vi "Initialize From Config.vi"(8 "error in":errorcluster, 9 "Module Configurations":refnum<class "TBM module configuration.lvclass">[](array[class]), 10 "Modules":refnum<class "TBM module execution interface.lvclass">[](array[class]), 11 "Engine Configuration":refnum<class "synchronous engine configuration.lvclass">) -> (0 "error out":errorcluster, 3 "Engine Data Out":T1={"Main Tag Data"={"Double"=[], "Single"=[], "I64"=[], "I32"=[], "I16"=[], "I8"=[], "U64"=[], "U32"=[], "U16"=[], "U8"=[], "Boolean"=[], "String"=[], "Array of Double"=[], "Array of Single"=[], "Array of I64"=[], "Array of I32"=[], "Array of I16"=[], "Array of I8"=[], "Array of U64"=[], "Array of U32"=[], "Array of U16"=[], "Array of U8"=[], "Array of Boolean"=[], "Array of String"=[]}, "Module Info"={"Tag Bus Modules"=[], "Input Method Indices"=[], "Process Method Indices"=[], "Output Method Indices"=[], "Input Transfer Specifications"=[], "Parameter Transfer Specifications"=[], "Result Transfer Specifications"=[], "Output Transfer Specifications"=[], "Module Errors"=[], "UID"=""}, "Safe State?"=FALSE, "engine timing source"=refnum, "Processor"=5000, "Priority"=-2, "dT"=0})   [LabVIEW 2014, in "synchronous engine runtime.lvclass"]
uses:
  synchronous engine runtime.lvclass
  Engine Data.ctl
  <vilib>/NI/Module Timing Source/timing source/TBM timing source.lvclass
  <vilib>/NI/Tag Bus/table/data table.ctl
  Module Execution Info.ctl
  <vilib>/NI/Tag Bus Module Framework/runtime/TBM module execution interface.lvclass
  Data Table with Transfer Spec.ctl
  <vilib>/NI/Tag Bus/table/transfer specification.ctl
  <vilib>/NI/Tag Bus/tag/Data Type.ctl
  Configuration/synchronous engine configuration.lvclass
  <vilib>/NI/Tag Bus Module Framework/module configuration/TBM module configuration.lvclass
  <vilib>/NI/Module Timing Source/usec timing source/usec timing source.lvclass
  Configuration/synchronous engine configuration.lvclass/synchronous engine configuration.ctl
  Engine Configuration/engine configuration.lvclass/engine configuration.ctl
  <vilib>/NI/Tag Bus/dictionary/data dictionary.lvclass/data dictionary.ctl
  <vilib>/NI/Configuration Framework/serializable configuration/NISE_CEF_serializable configuration.lvclass/NISE_CEF_serializable configuration.ctl
  <vilib>/NI/Configuration Framework/serializable configuration/Read UID.vi
  Configuration/Read Processor.vi
  Configuration/Read Priority.vi
  Configuration/Read Timing Source dt.vi
  <vilib>/Utility/LVClass/Get LV Class Name.vi
  <vilib>/NI/Configuration Framework/error generator/NISE_error generator.vi
  <vilib>/NI/Tag Bus/dictionary/data dictionary.lvclass
  Engine Configuration/engine configuration.lvclass
  <vilib>/NI/Tag Bus/table/data table.lvlib
  <vilib>/NI/Tag Bus/tag/tag descriptor.lvclass
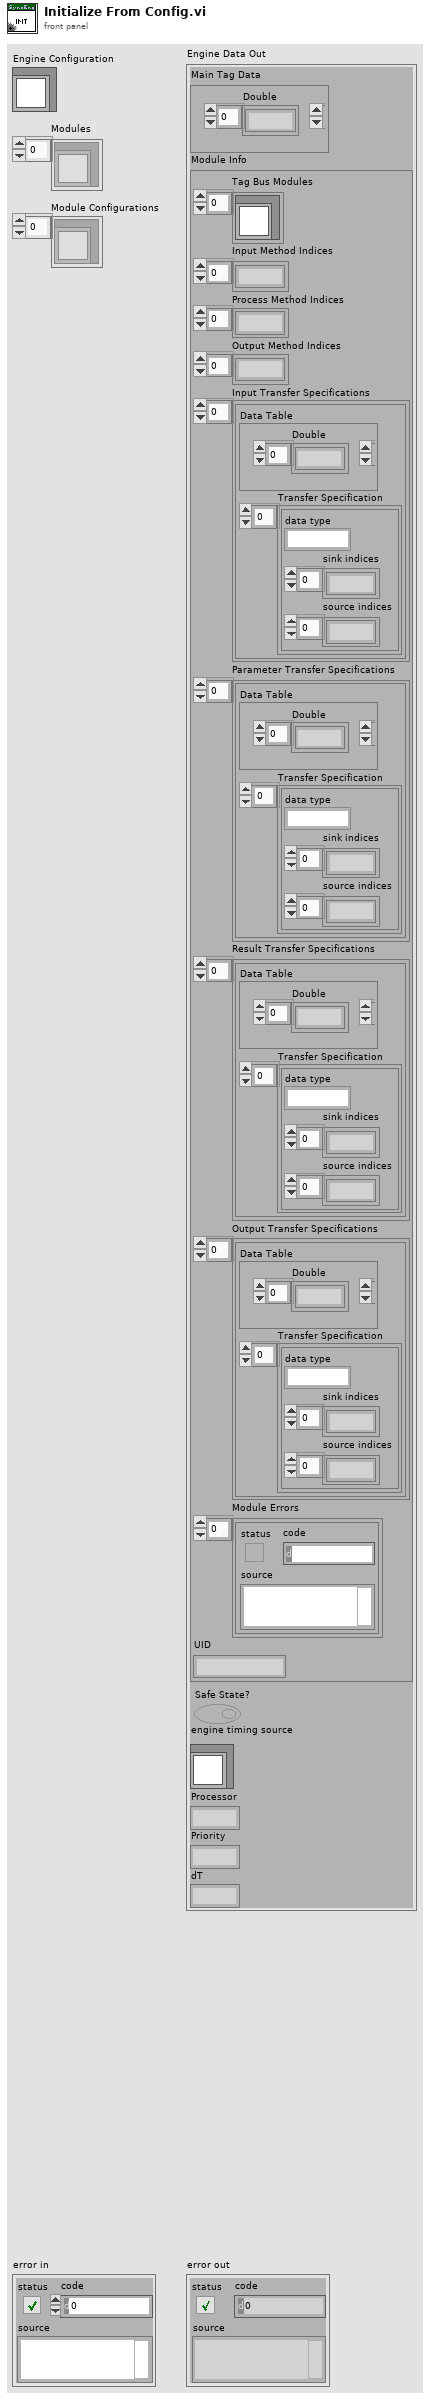
[diagram p1: front panel]
types:
  T1 = typedef "synchronous engine runtime.lvclass/Engine Data.ctl" = cluster{"Main Tag Data":T2, "Module Info":T3, "Safe State?":bool, "engine timing source":refnum<class "TBM timing source.lvclass">, "Processor":i32, "Priority":i32, "dT":u32}
  T2 = typedef "tag bus.lvlib/data table.lvlib/data table.ctl" = cluster{"Double":dbl[], "Single":sgl[], "I64":i64[], "I32":i32[], "I16":i16[], "I8":i8[], "U64":u64[], "U32":u32[], "U16":u16[], "U8":u8[], "Boolean":bool[], "String":string[], "Array of Double":cluster{"DBL Array":dbl[]}[], "Array of Single":cluster{"SGL Array":sgl[]}[], "Array of I64":cluster{"I64 Array":i64[]}[], "Array of I32":cluster{"I32 Array":i32[]}[], "Array of I16":cluster{"I16 Array":i16[]}[], "Array of I8":cluster{"I8 Array":i8[]}[], "Array of U64":cluster{"U64 Array":u64[]}[], "Array of U32":cluster{"U32 Array":u32[]}[], "Array of U16":cluster{"U16 Array":u16[]}[], "Array of U8":cluster{"U8 Array":u8[]}[], "Array of Boolean":cluster{"Boolean Array":bool[]}[], "Array of String":cluster{"String Array":string[]}[]}
  T3 = typedef "synchronous engine runtime.lvclass/Module Execution Info.ctl" = cluster{"Tag Bus Modules":refnum<class "TBM module execution interface.lvclass">[], "Input Method Indices":i32[], "Process Method Indices":i32[], "Output Method Indices":i32[], "Input Transfer Specifications":T4[], "Parameter Transfer Specifications":T4[], "Result Transfer Specifications":T4[], "Output Transfer Specifications":T4[], "Module Errors":errorcluster[], "UID":string}
  T4 = typedef "synchronous engine runtime.lvclass/Data Table with Transfer Spec.ctl" = cluster{"Data Table":T2, "Transfer Specification":T5[]}
  T5 = typedef "tag bus.lvlib/data table.lvlib/transfer specification.ctl" = cluster{"data type":T6, "sink indices":i32[], "source indices":i32[]}
  T6 = typedef "tag bus.lvlib/tag descriptor.lvclass/Data Type.ctl" = enum16{"Double", "Single", "I64", "I32", "I16", "I8", "U64", "U32", "U16", "U8", "Boolean", "String", "Array of Double", "Array of Single", "Array of I64", "Array of I32", "Array of I16", "Array of I8", "Array of U64", "Array of U32", "Array of U16", "Array of U8", "Array of Boolean", "Array of String"}
  T7 = typedef "TBM channel.lvclass/data tables.ctl" = cluster{"input data":T8, "processing parameter":T8, "processing result":T8, "output data":T8}
  T8 = typedef "tag bus.lvlib/dictionary table pair.ctl" = cluster{"data dictionary":refnum<class "data dictionary.lvclass">, "data table":T2}
  T9 = typedef "TBM module execution interface.lvclass/execution settings.ctl" = cluster{"reads inputs":bool, "processes data":bool, "writes outputs":bool}
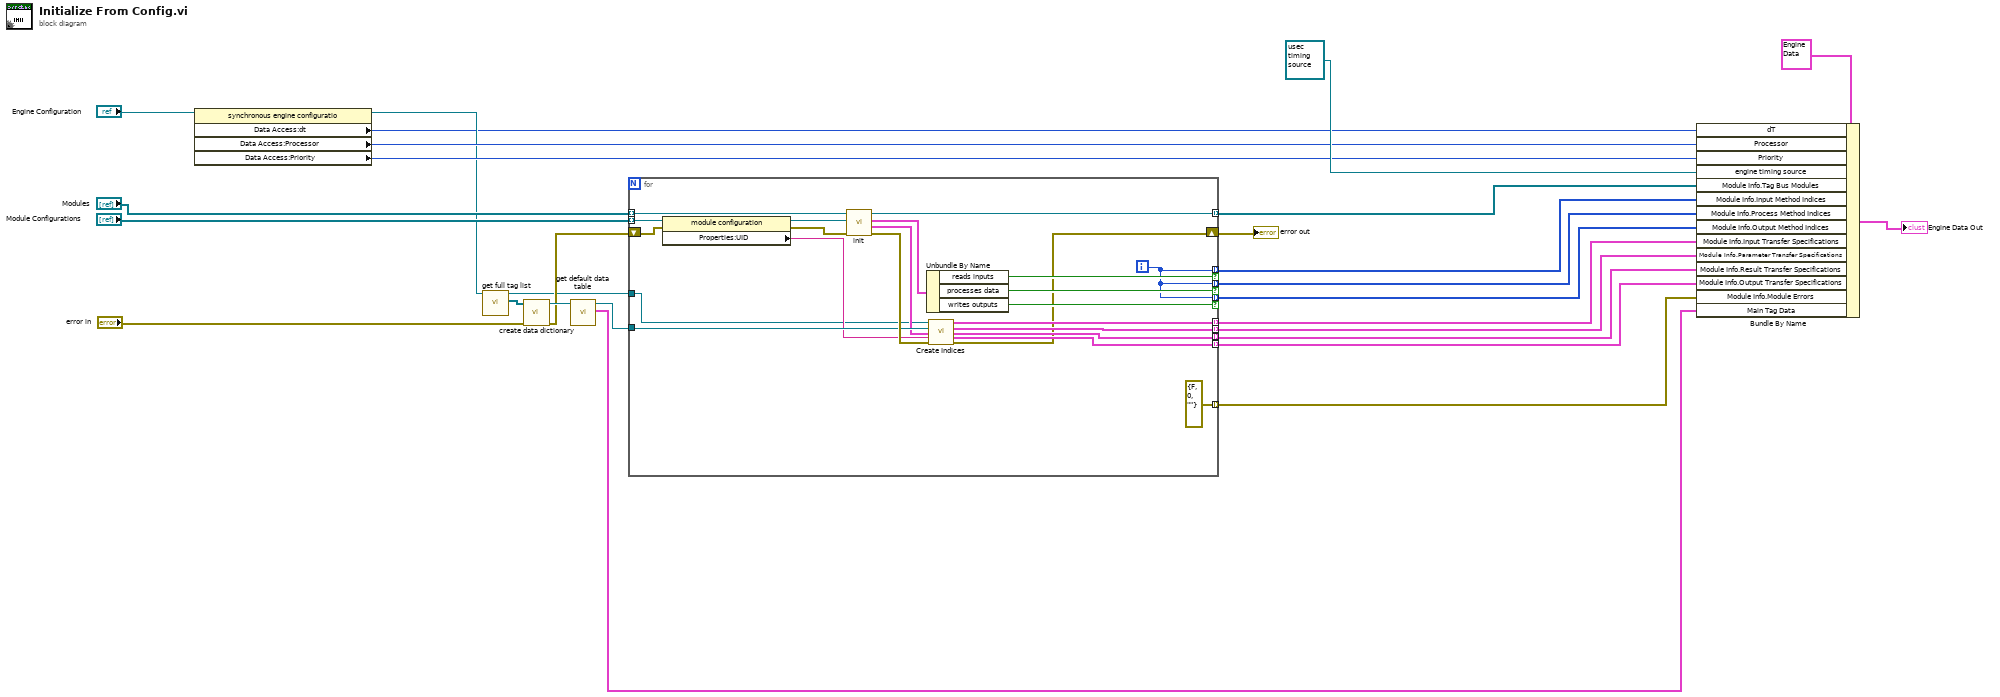
[diagram p0: block diagram]
diagram:
  n1 = property class="synchronous engine configuratio"(reference="Engine Configuration") -> (reference out=w2:refnum<class "synchronous engine configuration.lvclass">, "Data Access:dt"=w1:u32, "Data Access:Processor"=w4:i32, "Data Access:Priority"=w3:i32)  [unwired: 1 in, 1 out]
  n2 = call "get full tag list.vi"("engine configuration in"=w2) -> ("tag list"=w10:refnum<class "tag descriptor.lvclass">[], "engine configuration out"=w7:refnum<class "synchronous engine configuration.lvclass">)  [unwired: 9 in]
  n3 = call <vilib>:"create data dictionary.vi"("error in"="error in", "system tags"=w10) -> ("error out"=w8:errorcluster, "data dictionary"=w9:refnum<class "data dictionary.lvclass">)  [unwired: 8 in]
  n4 = call <vilib>:"get default data table.vi"("data dictionary in"=w9) -> ("default data table"=w16:T2, "data dictionary out"=w15:refnum<class "data dictionary.lvclass">)  [unwired: 9 in]
  n5 = for {
    tunnel: "Module Configurations" -> [w35] mode=indexing
    shift-right: [w30] -> w18
    shift-left: w8 -> [w32]
    tunnel: "Modules" -> [w49] mode=indexing
    tunnel: [w31] -> w27 mode=indexing
    tunnel: [w40] -> w25 mode=indexing if=w48
    tunnel: [w40] -> w24 mode=indexing if=w47
    tunnel: [w40] -> w23 mode=indexing if=w46
    tunnel: [w45] -> w22 mode=indexing
    tunnel: [w44] -> w21 mode=indexing
    tunnel: [w43] -> w20 mode=indexing
    tunnel: [w42] -> w19 mode=indexing
    tunnel: [errorcluster {"status"=FALSE, "code"=0, "source"=""} ("error constant")] -> w17 mode=indexing
    tunnel: w15 -> [w38]
    tunnel: w7 -> [w28]
    i -> [w40]
    n6 = property class="module configuration"(reference=w35, error in=w32) -> (reference out=w34:refnum<class "TBM module configuration.lvclass">, error out=w33:errorcluster, "Properties:UID"=w29:string)
    n7 = call-dynamic "init.vi"("error in"=w33, "module configuration"=w34, "module in"=w49) -> ("error out"=w41:errorcluster, "data allocations"=w36:T7, "execution settings"=w37:T9, "module out"=w31:refnum<class "TBM module execution interface.lvclass">)  [unwired: 5 in]
    n8 = Unbundle By Name(w37) -> ("reads inputs"=w48:bool, "processes data"=w47:bool, "writes outputs"=w46:bool)
    n9 = call "Create Indices.vi"("synchronous engine configuration"=w28, "main data dictionary"=w38, "data description"=w36, "Module ID"=w29, "error in"=w41) -> ("Input Transfer Specification"=w45:T4, "Parameter Transfer Specifcation"=w44:T4, "Result Transfer Specifcation"=w43:T4, "Output Transfer Specifcation"=w42:T4, "error out"=w30:errorcluster)  [unwired: 6 in]
  }
  "error out" <- w18
  n10 = Bundle By Name(cluster=T1 {"Main Tag Data"={"Double"=[], "Single"=[], "I64"=[], "I32"=[], "I16"=[], "I8"=[], "U64"=[], "U32"=[], "U16"=[], "U8"=[], "Boolean"=[], "String"=[], "Array of Double"=[], "Array of Single"=[], "Array of I64"=[], "Array of I32"=[], "Array of I16"=[], "Array of I8"=[], "Array of U64"=[], "Array of U32"=[], "Array of U16"=[], "Array of U8"=[], "Array of Boolean"=[], "Array of String"=[]}, "Module Info"={"Tag Bus Modules"=[], "Input Method Indices"=[], "Process Method Indices"=[], "Output Method Indices"=[], "Input Transfer Specifications"=[], "Parameter Transfer Specifications"=[], "Result Transfer Specifications"=[], "Output Transfer Specifications"=[], "Module Errors"=[], "UID"=""}, "Safe State?"=FALSE, "engine timing source"=refnum, "Processor"=0, "Priority"=0, "dT"=0} ("Engine Data"), "dT"=w1, "Processor"=w4, "Priority"=w3, "engine timing source"=refnum<class "usec timing source.lvclass"> refnum ("usec timing source.lvclass"), "Module Info.Tag Bus Modules"=w27, "Module Info.Input Method Indices"=w25, "Module Info.Process Method Indices"=w24, "Module Info.Output Method Indices"=w23, "Module Info.Input Transfer Specifications"=w22, "Module Info.Parameter Transfer Specifications"=w21, "Module Info.Result Transfer Specifications"=w20, "Module Info.Output Transfer Specifications"=w19, "Module Info.Module Errors"=w17, "Main Tag Data"=w16) -> (→"Engine Data Out":T1)
